vi "OnRequestReceived.vi"(4 "return":refnum<vi>, 5 "事件数据":T2, 6 "控件引用":refnum<k24>, 7 "事件通用数据":cluster{"事件源":i32, "事件类型":u32, "时间标识":u32}) -> (1 "事件数据输出":cluster{"return value":refnum<k24>})   [LabVIEW 2025]
uses:
  CFX_dll/CFX.dll
  ctl/CFX_data.ctl
  SubVI/table/1 model/a log/_myType runlog cmd.ctl
  <vilib>/regexp/Match Regular Expression.xnode
panel:
  out "CFX_Message_In":T1
  out "StrOut":string
  in  "error in":errorcluster caption="错误输入"
  out "error out":errorcluster caption="错误输出"
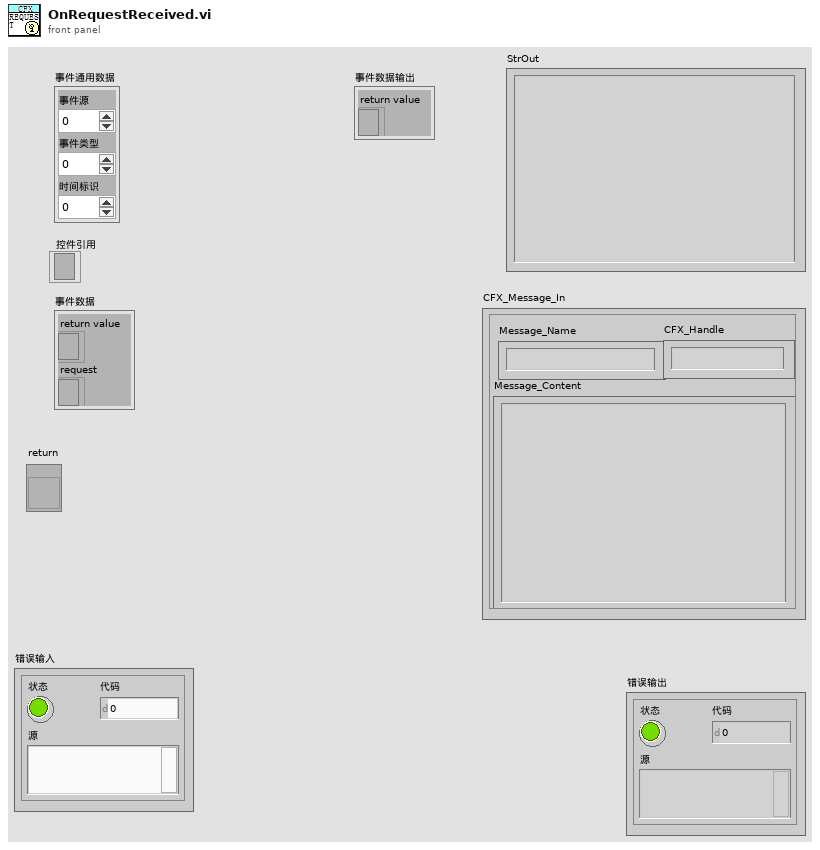
[diagram p1: front panel]
types:
  T1 = cluster{"Message_Name":string, "CFX_Handle":string, "Message_Content":string}
  T2 = cluster{"return value":refnum<k24>, "request":refnum<k24>}
  T3 = typedef "_myType runlog cmd.ctl" = enum16{"init", "push (-1: error)", "push (0: user)", "push (1: logical)", "push (2: driver)", "push (3: lib-core)", "push (4: reserved)", "pop", "more?"}
  T4 = cluster{"CFXHandle":string, "RequestNetworkUri":string, "RequestTargetAddress":string, "CFX_Message_In":cluster{"Message_Name":string, "Message_Content":string}, "CFX_Message_out":cluster{"Message_Name":string, "Message_Content":string}, "CFX_data":refnum<vi>}
  T5 = typedef "CFX_data.ctl" = cluster{"Vendor":string, "UniqueIdentifier":string, "FriendlyName":string, "ModelNumber":string, "SerialNumber":string, "NumberofLanes":string, "CodeIn":string, "CodeOut":string, "Unitldentifer":string, "PositionNumber":string, "PositionName":string, "OldState":string, "NewState":string, "OldStateDuration":string, "Faultcode":string, "Operatorldentifer":string, "LoginName":string, "RecipeName":string, "Revision":string, "Activate formula":string, "Description":string}
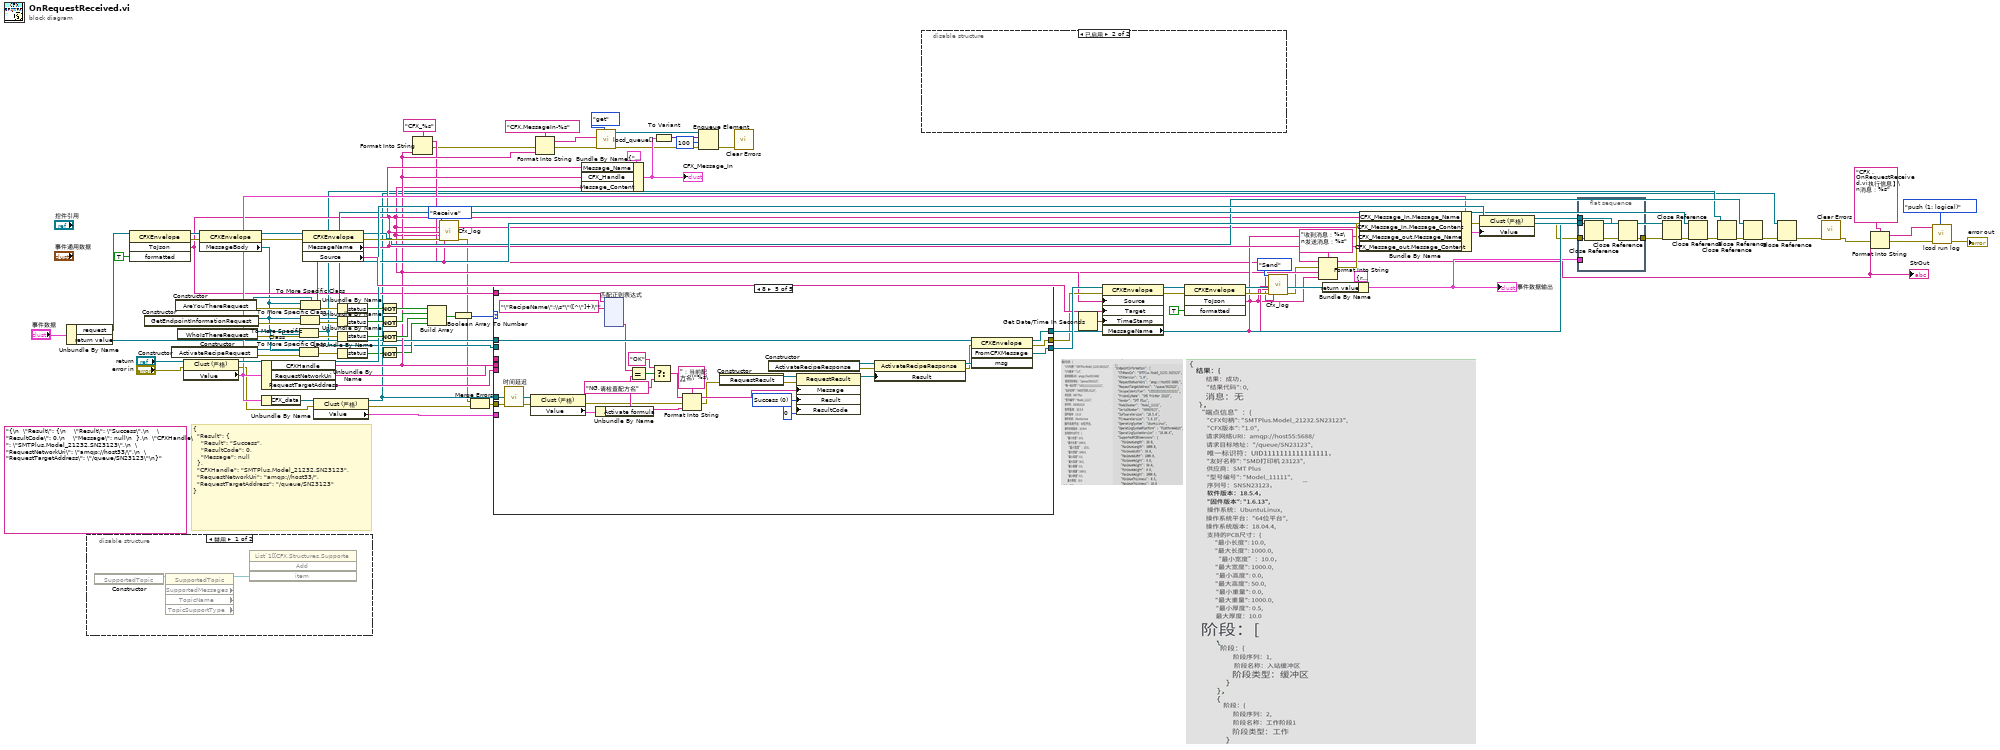
[diagram p0: block diagram]
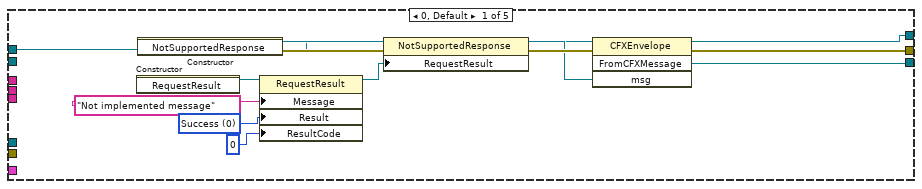
[diagram p3: hidden frame]
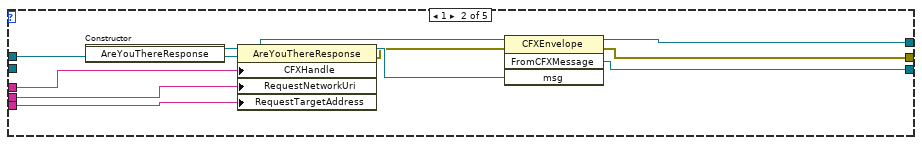
[diagram p4: hidden frame]
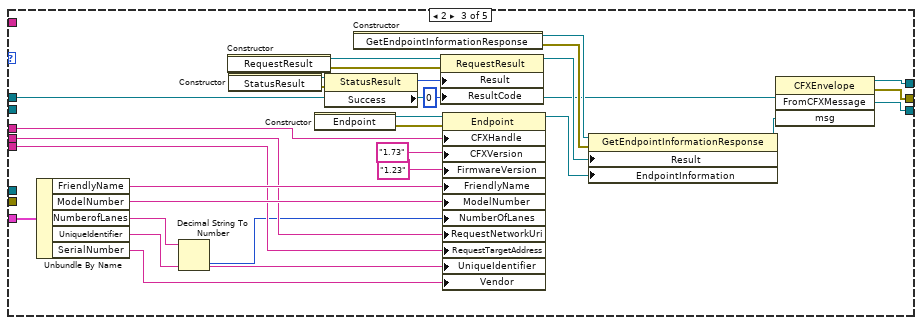
[diagram p5: hidden frame]
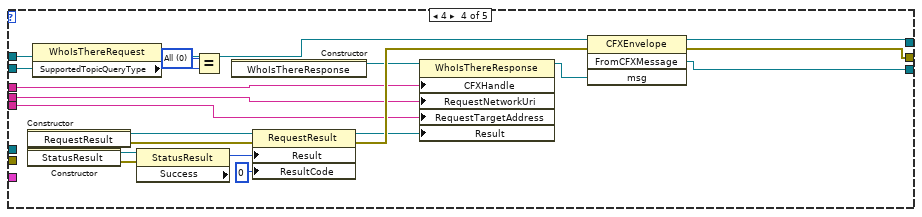
[diagram p6: hidden frame]
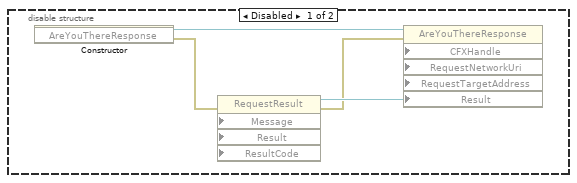
[diagram p7: hidden frame]
diagram:
  (unwired) "{\n  \"Result\": {\n    \"Result\": \"Success\",\n    \"ResultCode\": 0,\n    \"Message\": null\n  },\n  \"CFXHandle\": \"SMTPlus.Model_21232.SN23123\",\n  \"RequestNetworkUri\": \"amqp://host33/\",\n  \"RequestTargetAddress\": \"/queue/SN23123\"\n}" ("Message")
  # "{\n  \"Result\": {\n    \"Result\": \"Success\",\n    \"ResultCode\": 0,\n    \"Message\": null\n  },\n  \"CFXHandle\": \"SMTPlus.Model_21232.SN23123\",\n  \"RequestNetworkUri\": \"amqp://host33/\",\n  \"RequestTargetAddress\": \"/queue/SN23123\"\n}"
  n1 = Unbundle By Name("事件数据") -> ("request"=w51:refnum<k24>, "return value"=w20:refnum<k24>)
  n2 = disable-structure shown="禁用" {
    frame Disabled {
      n3 = constructor class="SupportedTopic"() -> (reference out=w102:refnum<k24>)  [unwired: 3 in, 2 out]
      n4 = property on="属性节点" class="SupportedTopic" props=["SupportedMessages", "TopicName", "TopicSupportType"](reference=w102) -> (reference out=w101:refnum<k24>)  [unwired: 1 in, 4 out]
      n5 = invoke class="List`1[[CFX.Structures.Supporte" method="Add"("item"=w101) -> ()  [unwired: 3 in, 4 out]
    }
    frame Enabled {
    }
  }
  n6 = invoke on="调用节点" class="CFXEnvelope" method="ToJson"(reference=w51, "formatted"=TRUE) -> (reference out=w57:refnum<k24>, error out=w55:errorcluster, "ToJson"=w11:string)  [unwired: 2 in, 1 out]
  n7 = constructor class="GetEndpointInformationRequest"() -> (reference out=w84:refnum<k24>, error out=w52:errorcluster)  [unwired: 3 in, 1 out]
  n8 = constructor class="ActivateRecipeRequest"() -> (reference out=w9:refnum<k24>, error out=w18:errorcluster)  [unwired: 3 in, 1 out]
  n9 = constructor class="AreYouThereRequest"() -> (reference out=w89:refnum<k24>, error out=w88:errorcluster)  [unwired: 3 in, 1 out]
  n10 = constructor class="WhoIsThereRequest"() -> (reference out=w19:refnum<k24>, error out=w83:errorcluster)  [unwired: 3 in, 1 out]
  n11 = property class="Clust (严格)"(reference="return", error in="error in") -> (reference out=w77:refnum<vi>, error out=w4:errorcluster, "Value"=w47:T4)
  n12 = property class="CFXEnvelope"(reference=w57, error in=w55) -> (reference out=w98:refnum<k24>, error out=w94:errorcluster, "MessageBody"=w10:refnum<k24>)
  n13 = Unbundle By Name(w47) -> ("CFX_data"=w46:refnum<vi>)
  n14 = Unbundle By Name(w47) -> ("CFXHandle"=w25:string, "RequestNetworkUri"=w97:string, "RequestTargetAddress"=w96:string)
  n15 = To More Specific Class(target class=w19, reference=w10, error in=w83) -> (specific class reference=w8:refnum<k24>, error out=w82:errorcluster)
  n16 = To More Specific Class(target class=w9, reference=w10, error in=w18) -> (error out=w17:errorcluster)  [unwired: 1 out]
  n17 = To More Specific Class(target class=w84, reference=w10, error in=w52) -> (specific class reference=w71:refnum<k24>, error out=w86:errorcluster)
  n18 = To More Specific Class(target class=w89, reference=w10, error in=w88) -> (specific class reference=w73:refnum<k24>, error out=w74:errorcluster)
  n19 = property on="属性节点" class="CFXEnvelope"(reference=w98, error in=w94) -> (reference out=w53:refnum<k24>, error out=w54:errorcluster, "MessageName"=w40:string, "Source"=w92:string)
  n20 = property class="Clust (严格)"(reference=w46, error in=w4) -> (reference out=w7:refnum<vi>, error out=w2:errorcluster, "Value"=w49:T5)
  n21 = Unbundle By Name(w74) -> ("status"=w87:bool)
  n22 = Unbundle By Name(w86) -> ("status"=w85:bool)
  n23 = Unbundle By Name(w82) -> ("status"=w81:bool)
  n24 = Unbundle By Name(w17) -> ("status"=w16:bool)
  n25 = Not(x=w87) -> (.not. x?=w80:bool)
  n26 = Not(x=w85) -> (.not. x?=w79:bool)
  n27 = Not(x=w81) -> (.not. x?=w78:bool)
  n28 = Not(x=w16) -> (.not. x?=w15:bool)
  n29 = Format Into String(format string="CFX_%s" ("log_path"), w25) -> (resulting string=w24:string, error out=w21:errorcluster)  [unwired: 2 in]
  n30 = Build Array(w80, w79, w78, w15) -> (w91:bool[])
  n31 = call "Cfx_log.vi"("R/W"=enum16{"Send", "Receive"}."Receive", "Message_Name"=w40, "Message_Content"=w11, "error in"=w54, "log_path"=w24) -> ("error out"=w6:errorcluster)  [unwired: 13 in, 1 out]
  n32 = Boolean Array To Number(Boolean array=w91) -> (number=w90:u32)
  n33 = Merge Errors(w6, w2) -> (w3:errorcluster)
  n34 = case shown="8" w90 {
    tunnel: [w110 w122 w154 w166 w202] -> w99
    tunnel: w97 -> [_ w117 w130 w159 _]
    tunnel: w96 -> [_ w116 w129 w158 _]
    tunnel: w25 -> [_ w125 w131 w160 _]
    tunnel: w20 -> [w111 w124 w127 w174 w203]
    tunnel: [w109 w121 w153 w157 w201] -> w69
    tunnel: [w108 w120 w152 w156 w200] -> w68
    tunnel: w49 -> [_ _ w132 _ _]
    tunnel: w8 -> [_ _ _ w155 _]
    tunnel: w11 -> [_ _ _ _ w188]
    tunnel: w3 -> [_ _ _ _ w177]
    tunnel: w7 -> [_ _ _ _ w180]
    frame 0, Default {
      w105 = 0 items=["Success", "PartialSuccess", "Failed", "Warning"] ("Result")
      n35 = constructor class="RequestResult"() -> (reference out=w107:refnum<k24>)  [unwired: 3 in, 2 out]
      n36 = constructor class="NotSupportedResponse"() -> (reference out=w115:refnum<k24>, error out=w114:errorcluster)  [unwired: 3 in, 1 out]
      n37 = property on="属性节点" class="RequestResult"(reference=w107, "Message"="Not implemented message", "Result"=w105, "ResultCode"=0) -> (reference out=w106:refnum<k24>)  [unwired: 1 in, 1 out]
      n38 = property class="NotSupportedResponse"(reference=w115, error in=w114, "RequestResult"=w106) -> (reference out=w112:refnum<k24>, error out=w113:errorcluster)
      n39 = invoke class="CFXEnvelope" method="FromCFXMessage"(reference=w111, error in=w113, "msg"=w112) -> (reference out=w109:refnum<k24>, error out=w108:errorcluster, "FromCFXMessage"=w110:refnum<k24>)  [unwired: 1 in, 1 out]
    }
    frame 1 {
      n40 = constructor class="AreYouThereResponse"() -> (reference out=w118:refnum<k24>)  [unwired: 3 in, 2 out]
      n41 = property class="AreYouThereResponse"(reference=w118, "CFXHandle"=w125, "RequestNetworkUri"=w117, "RequestTargetAddress"=w116) -> (reference out=w123:refnum<k24>, error out=w119:errorcluster)  [unwired: 1 in]
      n42 = invoke class="CFXEnvelope" method="FromCFXMessage"(reference=w124, error in=w119, "msg"=w123) -> (reference out=w121:refnum<k24>, error out=w120:errorcluster, "FromCFXMessage"=w122:refnum<k24>)  [unwired: 1 in, 1 out]
    }
    frame 2 {
      n43 = Unbundle By Name(w132) -> ("FriendlyName"=w147:string, "ModelNumber"=w148:string, "NumberofLanes"=w149:string, "UniqueIdentifier"=w150:string, "SerialNumber"=w151:string)
      n44 = Decimal String To Number(string=w149) -> (number=w126:i32)  [unwired: 2 in, 1 out]
      n45 = constructor class="RequestResult"() -> (reference out=w138:refnum<k24>, error out=w139:errorcluster)  [unwired: 3 in, 1 out]
      n46 = constructor class="StatusResult"() -> (reference out=w140:refnum<k24>, error out=w141:errorcluster)  [unwired: 3 in, 1 out]
      n47 = constructor class="Endpoint"() -> (reference out=w146:refnum<k24>, error out=w143:errorcluster)  [unwired: 3 in, 1 out]
      n48 = property class="StatusResult"(reference=w140, error in=w141) -> ("Success"=w142:i32)  [unwired: 2 out]
      n49 = constructor class="GetEndpointInformationResponse"() -> (reference out=w137:refnum<k24>, error out=w136:errorcluster)  [unwired: 3 in, 1 out]
      n50 = property on="属性节点" class="RequestResult"(reference=w138, error in=w139, "Result"=w142, "ResultCode"=0) -> (reference out=w144:refnum<k24>)  [unwired: 1 out]
      n51 = property class="Endpoint"(reference=w146, error in=w143, "CFXHandle"=w131, "CFXVersion"="1.73", "FirmwareVersion"="1.23", "FriendlyName"=w147, "ModelNumber"=w148, "NumberOfLanes"=w126, "RequestNetworkUri"=w130, "RequestTargetAddress"=w129, "UniqueIdentifier"=w150, "Vendor"=w151) -> (reference out=w145:refnum<k24>)  [unwired: 1 out]
      n52 = property class="GetEndpointInformationResponse"(reference=w137, error in=w136, "Result"=w144, "EndpointInformation"=w145) -> (reference out=w128:refnum<k24>)  [unwired: 1 out]
      n53 = invoke class="CFXEnvelope" method="FromCFXMessage"(reference=w127, "msg"=w128) -> (reference out=w153:refnum<k24>, error out=w152:errorcluster, "FromCFXMessage"=w154:refnum<k24>)  [unwired: 2 in, 1 out]
    }
    frame 4 {
      w165 = 0 items=["All", "Any", "Ignore"] ("SupportedTopicQueryType")
      n54 = constructor class="RequestResult"() -> (reference out=w173:refnum<k24>, error out=w172:errorcluster)  [unwired: 3 in, 1 out]
      n55 = constructor class="StatusResult"() -> (reference out=w170:refnum<k24>, error out=w169:errorcluster)  [unwired: 3 in, 1 out]
      n56 = property class="WhoIsThereRequest"(reference=w155) -> ("SupportedTopicQueryType"=w164:i32)  [unwired: 1 in, 2 out]
      n57 = property class="StatusResult"(reference=w170, error in=w169) -> ("Success"=w168:i32)  [unwired: 2 out]
      n58 = Equal?(x=w165, y=w164) -> ()  [unwired: 1 out]
      n59 = constructor class="WhoIsThereResponse"() -> (reference out=w163:refnum<k24>)  [unwired: 3 in, 2 out]
      n60 = property on="属性节点" class="RequestResult"(reference=w173, error in=w172, "Result"=w168, "ResultCode"=0) -> (reference out=w162:refnum<k24>, error out=w171:errorcluster)
      n61 = property on="属性节点" class="WhoIsThereResponse"(reference=w163, "CFXHandle"=w160, "RequestNetworkUri"=w159, "RequestTargetAddress"=w158, "Result"=w162) -> (reference out=w161:refnum<k24>)  [unwired: 1 in, 1 out]
      n62 = invoke class="CFXEnvelope" method="FromCFXMessage"(reference=w174, error in=w171, "msg"=w161) -> (reference out=w157:refnum<k24>, error out=w156:errorcluster, "FromCFXMessage"=w166:refnum<k24>)  [unwired: 1 in, 1 out]
    }
    frame 8 {
      w194 = 0 items=["Success", "PartialSuccess", "Failed", "Warning"] ("Result")
      n63 = call "时间延迟"("error in (no error)"=w177) -> ("error out"=w179:errorcluster)  [unwired: 10 in]
      n64 = property class="Clust (严格)"(reference=w180, error in=w179) -> (error out=w176:errorcluster, "Value"=w178:T5)  [unwired: 1 out]
      n65 = Unbundle By Name(w178) -> ("Activate formula"=w181:string)
      n66 = xnode "匹配正则表达式"("输入字符串"=w188, "正则表达式"="\"RecipeName\":\\s*\"([^\"]+)\"") -> ("子匹配 1"=w186:string)  [unwired: 4 in, 5 out]
      n67 = Equal?(x=w186, y=w181) -> (x = y?=w185:bool)
      n68 = Select(t="OK", s=w185, f="NG,请检查配方名") -> (s? t:f=w182:string)
      n69 = Format Into String(format string="：当前配方名\"%s\"" ("格式字符串"), initial string=w182, error in=w176, w181) -> (resulting string=w190:string, error out=w189:errorcluster)
      n70 = constructor class="RequestResult"(error in=w189) -> (reference out=w197:refnum<k24>, error out=w196:errorcluster)  [unwired: 2 in, 1 out]
      n71 = constructor class="ActivateRecipeResponse"() -> (reference out=w199:refnum<k24>, error out=w198:errorcluster)  [unwired: 3 in, 1 out]
      n72 = property class="RequestResult"(reference=w197, error in=w196, "Message"=w190, "Result"=w194, "ResultCode"=0) -> (reference out=w195:refnum<k24>)  [unwired: 1 out]
      n73 = property on="属性节点" class="ActivateRecipeResponse"(reference=w199, error in=w198, "Result"=w195) -> (reference out=w192:refnum<k24>, error out=w175:errorcluster)
      n74 = invoke class="CFXEnvelope" method="FromCFXMessage"(reference=w203, error in=w175, "msg"=w192) -> (reference out=w201:refnum<k24>, error out=w200:errorcluster, "FromCFXMessage"=w202:refnum<k24>)  [unwired: 1 in, 1 out]
    }
  }
  n75 = Format Into String(format string="CFX.MessageIn-%s" ("格式字符串"), error in=w21, w25) -> (resulting string=w44:string, error out=w36:errorcluster)  [unwired: 1 in]
  n76 = Bundle By Name(cluster=T1 {"Message_Name"="", "CFX_Handle"="", "Message_Content"=""} ("CFX_Message_In"), "Message_Name"=w40, "CFX_Handle"=w25, "Message_Content"=w11) -> (w38:T1)
  "CFX_Message_In" <- w38
  n77 = call "locd_queue[].vi"("cmd"=enum16{"init", "get", "set", "end"}."get", "error in"=w36, "queue_name"=w44) -> ("error out"=w35:errorcluster, "queue_out"=w42:refnum<queue>)  [unwired: 4 in, 3 out]
  n78 = To Variant(anything=w38) -> (Variant=w39:variant)
  n79 = Enqueue Element(queue=w42, element=w39, timeout in ms (-1)=100 ("超时毫秒(-1)"), error in (no error)=w35) -> (error out=w22:errorcluster)  [unwired: 2 out]
  n80 = call <vilib>:"Clear Errors.vi"("error in (no error)"=w22) -> ()  [unwired: 5 in, 2 out]
  n81 = disable-structure shown="已启用" {
    frame Disabled {
      n82 = constructor class="AreYouThereResponse"() -> (reference out=w326:refnum<k24>, error out=w324:errorcluster)  [unwired: 3 in, 1 out]
      n83 = property class="RequestResult" props=["Message", "Result", "ResultCode"](error in=w324) -> (reference out=w325:refnum<k24>, error out=w323:errorcluster)  [unwired: 4 in]
      n84 = property class="AreYouThereResponse" props=["CFXHandle", "RequestNetworkUri", "RequestTargetAddress", "Result"](reference=w326, error in=w323, "Result"=w325) -> ()  [unwired: 3 in, 2 out]
    }
    frame Enabled {
    }
  }
  n85 = Get Date/Time In Seconds() -> (seconds since 1Jan1904=w64:timestamp)
  n86 = property on="属性节点" class="CFXEnvelope"(reference=w99, error in=w68, "Source"=w25, "Target"=w92, "TimeStamp"=w64) -> (reference out=w63:refnum<k24>, error out=w59:errorcluster, "MessageName"=w28:string)
  n87 = invoke on="调用节点" class="CFXEnvelope" method="ToJson"(reference=w63, "formatted"=TRUE) -> (reference out=w60:refnum<k24>, "ToJson"=w27:string)  [unwired: 2 in, 2 out]
  n88 = call "Cfx_log.vi"("R/W"=enum16{"Send", "Receive"}."Send", "Message_Name"=w28, "Message_Content"=w27, "error in"=w59, "log_path"=w24) -> ("error out"=w1:errorcluster)  [unwired: 13 in, 1 out]
  n89 = Format Into String(format string="收到消息：%s\n发送消息：%s" ("格式字符串"), initial string=w40, error in=w1, w11, w27) -> (resulting string=w30:string, error out=w76:errorcluster)
  "StrOut" <- w30
  n90 = Bundle By Name(cluster=cluster{"return value":refnum<k24>} {"return value"=refnum} ("事件数据输出"), "return value"=w60) -> (w61:cluster{"return value":refnum<k24>})
  "事件数据输出" <- w61
  n91 = Bundle By Name(cluster=w47, "CFX_Message_In.Message_Name"=w40, "CFX_Message_In.Message_Content"=w11, "CFX_Message_out.Message_Name"=w28, "CFX_Message_out.Message_Content"=w27) -> (w50:T4)
  n92 = property class="Clust (严格)"(reference=w77, error in=w76, "Value"=w50) -> (reference out=w66:refnum<vi>, error out=w67:errorcluster)
  n93 = flat-sequence {
    tunnel: w69 -> [w331]
    tunnel: w67 -> [w330]
    tunnel: w66 -> [w328]
    tunnel: [w327] -> w23
    tunnel: w61 -> [_]
    frame #0 {
      n94 = Close Reference(reference=w331, error in (no error)=w330) -> (error out=w329:errorcluster)
      n95 = Close Reference(reference=w328, error in (no error)=w329) -> (error out=w327:errorcluster)
    }
  }
  n96 = Close Reference(reference=w73, error in (no error)=w23) -> (error out=w72:errorcluster)
  n97 = Close Reference(reference=w71, error in (no error)=w72) -> (error out=w70:errorcluster)
  n98 = Close Reference(reference=w8, error in (no error)=w70) -> (error out=w62:errorcluster)
  n99 = Close Reference(reference=w53, error in (no error)=w62) -> (error out=w14:errorcluster)
  n100 = Close Reference(reference=w7, error in (no error)=w14) -> (error out=w13:errorcluster)
  n101 = call <vilib>:"Clear Errors.vi"("error in (no error)"=w13) -> ("error out"=w12:errorcluster)  [unwired: 5 in, 1 out]
  n102 = Format Into String(format string="CFX .OnRequestReceived.vi执行信息】\n消息：%s", error in=w12, w30) -> (resulting string=w33:string, error out=w34:errorcluster)  [unwired: 1 in]
  n103 = call "lcod run log.vi"("cmd"=_myType_runlog_cmd."push (1: logical)", "Error In"=w34, "str in"=w33) -> ("Error Out"=→"error out":errorcluster)  [unwired: 6 in, 2 out]
